vi "Pixelfly Example to Delete.vi"() -> ()   [LabVIEW 2016]
doc: "A short program to demonstrate the fundamentals of control and image acquision with the pco.camera series. The program records a sequence of images, with \"live\" updating, until the \"StopRecording\" button is pressed. Use ctrl-H for more help on the individual controls and indicators.\n\nCopyright 2004, 2010 The Cooke Corporation."
uses:
  pco.sdk/CameraAccess/CameraAccess.lvlib
  pco.sdk/ImageSensor/ImageSensor.lvlib
  pco.sdk/TimingControl/TimingControl.lvlib
  pco.recorder/Recorder.lvlib
  pco.sdk/RecordingControl/RecordingControl.lvlib
  pco.sdk/CameraDescription/CameraDescription.lvlib
panel:
  out "Recorded Images":u32=298
  in  "TriggerMode":u16(ring) items=["auto sequence"=0, "software trigger"=1, "external exposure start & software trigger"=2, "external exposure control"=3, "external synchronized"=4, "fast external exposure control"=5, "external CDS control"=6, "slow external exposure control"=7, "external synchronized HDSDI"=258]
  in  "Quit":bool
  out "Image":u16[][](graph)
  in  "Start Record":bool
  out "Recording On":bool
  in  "roiY1":u16=2048 min=2 max=2048 step=1
  in  "roiX1":u16=2048 min=2 max=2048 step=1
  in  "roiY0":u16=1 min=1 max=2047 step=1
  in  "roiX0":u16=1 min=1 max=2047 step=1
  out "Image Height":u16=2048
  out "Image Width":u16=2048
  in  "dwImgCount":u32=10 caption="Required Number of Images" max=5304
  in  "DelayTimeBase":u16(ring)=2 items=["nanoseconds", "microseconds", "milliseconds"]
  in  "ExposureTimeBase":u16(ring)=2 items=["nanoseconds", "microseconds", "milliseconds"]
  in  "Exposure":u32=100 min=1
  in  "Delay":u32
  in  "Rate":i32(ring) items=["Low", "High"]
  # "Camera Setup"
  # "Parameters for image readout"
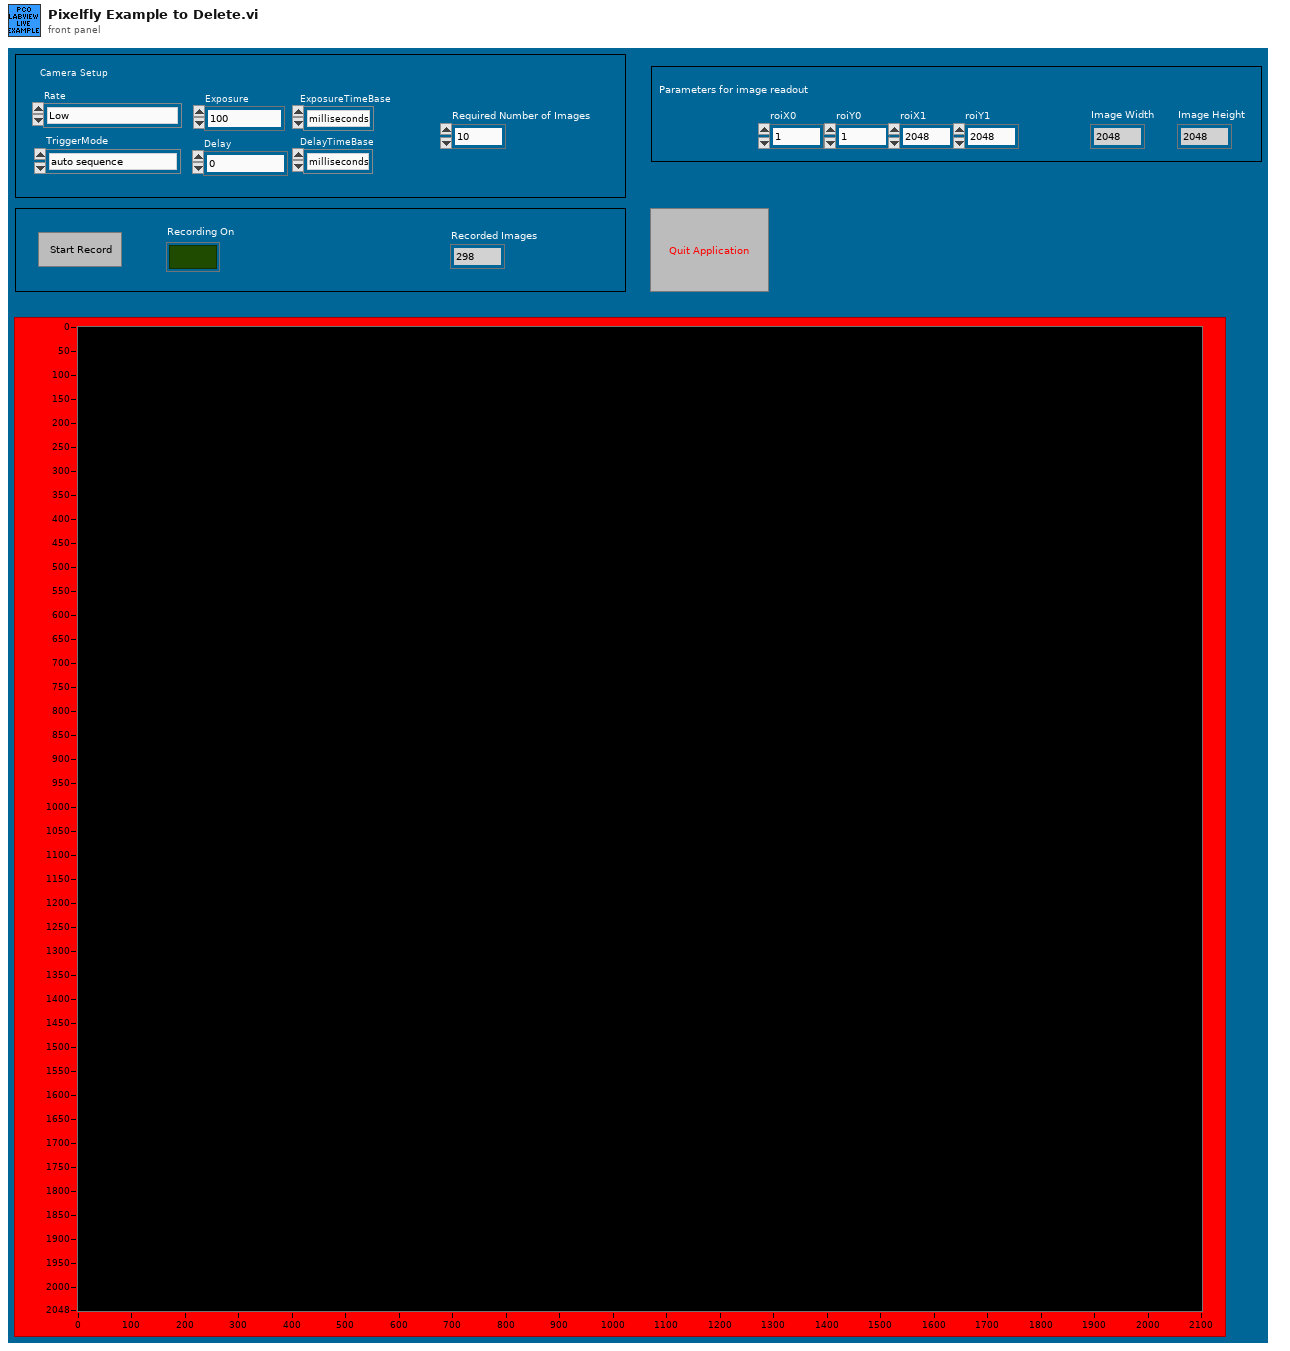
[diagram p1: front panel]
types:
  T1 = enum8{"Enabled", "Disabled", "Disabled and Grayed Out"}
  T2 = cluster{"wSensorTypeDESC":u16, "wSensorSubTypeDESC":u16, "wMaxHorzResStdDESC":u16, "wMaxVertResStdDESC":u16, "wMaxHorzResExtDESC":u16, "wMaxVertResExtDESC":u16, "wDynResDESC":u16, "wMaxBinHorzDESC":u16, "wBinHorzSteppingDESC":u16, "wMaxBinVertDESC":u16, "wBinVertSteppingDESC":u16, "wRoiHorStepsDESC":u16, "wRoiVertStepsDESC":u16, "wNumADCsDESC":u16, "wMinSizeHorzDESC":u16, "dwPixelRateDESC":u32[], "wConvFactDESC":u16[], "sCoolingSetpoints":i16[], "wSoftRoiHorStepsDESC":u16, "wSoftRoiVertStepsDESC":u16, "wIRDESC":u16, "wMinSizeVertDESC":u16, "dwMinDelayDESC":u32, "dwMaxDelayDESC":u32, "dwMinDelayStepDESC":u32, "dwMinExposureDESC":u32, "dwMaxExposureDESC":u32, "dwMinExposureStepDESC":u32, "dwMinDelayIRDESC":u32, "dwMaxDelayIRDESC":u32, "dwMinExposureIRDESC":u32, "dwMaxExposureIRDESC":u32, "wTimeTableDESC":u16, "wDoubleImageDESC":u16, "sMinCoolSetDESC":i16, "sMaxCoolSetDESC":i16, "sDefaultCoolSetDESC":i16, "wPowerDownModeDESC":u16, "wOffsetRegulationDESC":u16, "wColorPatternDESC":u16, "wPatternTypeDESC":u16, "wNumCoolingSetpoints":u16, "dwGeneralCapsDESC1":u32, "dwGeneralCapsDESC2":u32, "dwExtSyncFrequency":u32[], "dwGeneralCapsDESC3":u32, "dwGeneralCapsDESC4":u32}
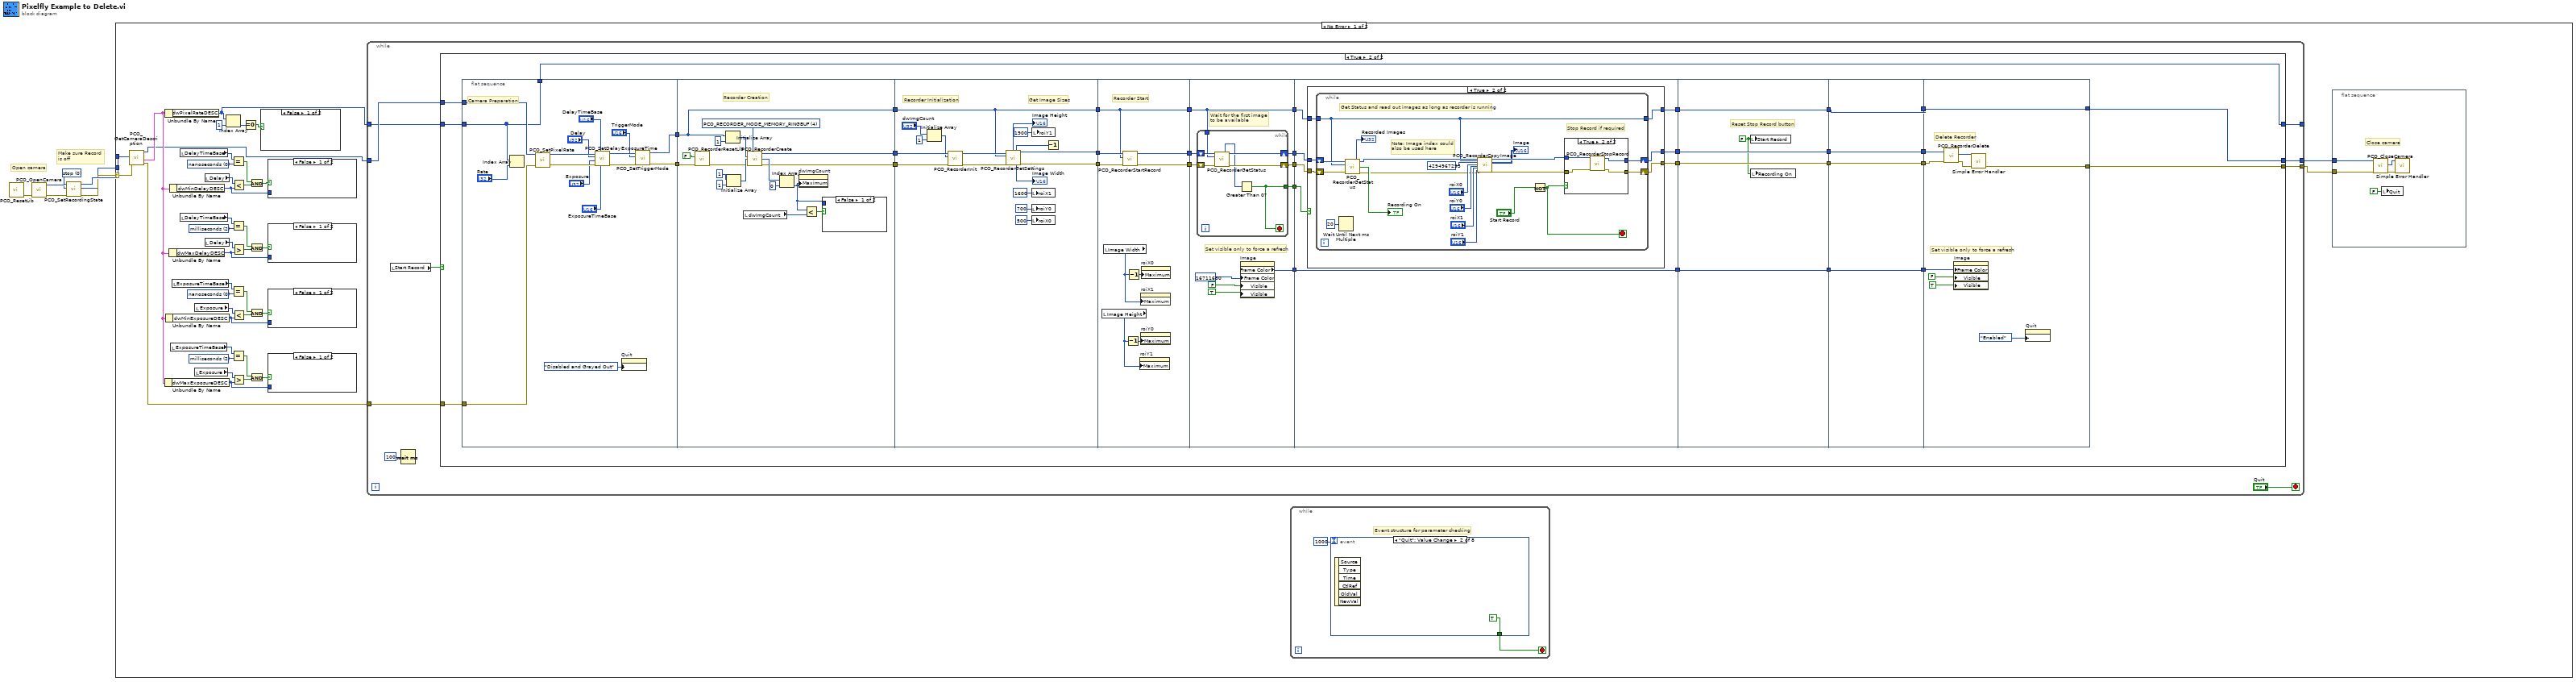
[diagram p0: block diagram]
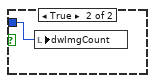
[diagram p3: hidden frame]
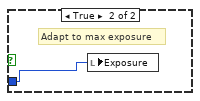
[diagram p6: hidden frame]
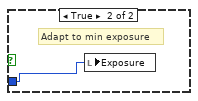
[diagram p7: hidden frame]
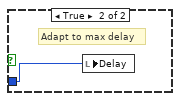
[diagram p8: hidden frame]
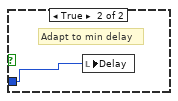
[diagram p9: hidden frame]
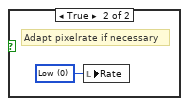
[diagram p10: hidden frame]
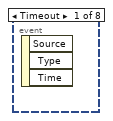
[diagram p11: hidden frame]
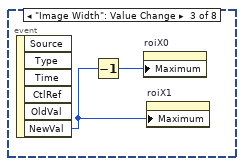
[diagram p12: hidden frame]
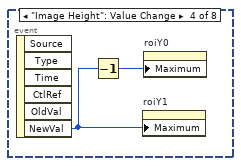
[diagram p13: hidden frame]
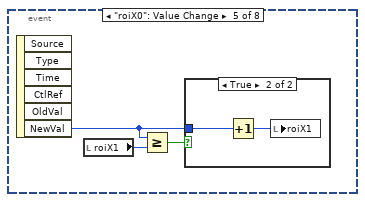
[diagram p14: hidden frame]
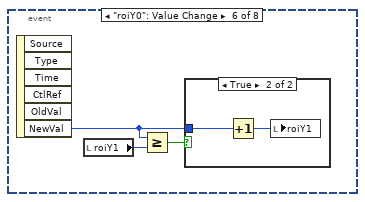
[diagram p16: hidden frame]
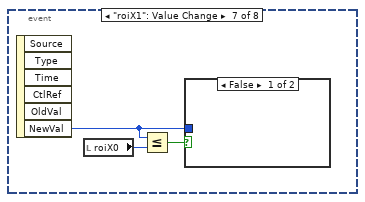
[diagram p18: hidden frame]
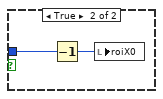
[diagram p19: hidden frame]
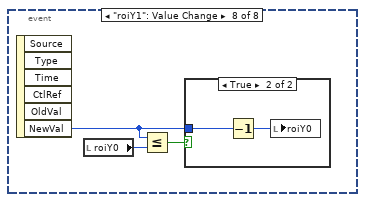
[diagram p20: hidden frame]
diagram:
  w4 = u16 0 items=["stop", "run"] ("wRecState")
  # "Make sure Record \nis off"
  # "Open camera"
  n1 = call "PCO_ResetLib.vi"() -> ("error out"=w7:errorcluster)  [unwired: 10 in, 1 out]
  n2 = call "PCO_OpenCamera.vi"("error in (no error)"=w7) -> ("error out"=w6:errorcluster, "ph out"=w5:u64)  [unwired: 8 in, 1 out]
  n3 = call "PCO_SetRecordingState.vi"("error in (no error)"=w6, "wRecState"=w4, "ph"=w5) -> ("error out"=w2:errorcluster, "ErrorMessage"=w1:i32, "ph out"=w3:u64)  [unwired: 6 in]
  n4 = case shown="No Error" w2 {
    selector: w2 -> [w14 w270]
    tunnel: w3 -> [w12 _]
    tunnel: w1 -> [_ w269]
    frame No Error {
      w35 = u16 2 items=["nanoseconds", "microseconds", "milliseconds"] ("DelayTimeBase")
      w44 = u16 0 items=["nanoseconds", "microseconds", "milliseconds"] ("DelayTimeBase")
      w28 = u16 2 items=["nanoseconds", "microseconds", "milliseconds"] ("DelayTimeBase")
      w19 = u16 0 items=["nanoseconds", "microseconds", "milliseconds"] ("DelayTimeBase")
      n5 = call "PCO_GetCameraDescription.vi"("error in (no error)"=w14, "ph"=w12) -> ("error out"=w13:errorcluster, "strDescription"=w46:T2, "ph out"=w11:u64)  [unwired: 6 in, 1 out]
      n6 = Unbundle By Name(w46) -> ("dwMaxExposureDESC"=w32:u32)
      n7 = Unbundle By Name(w46) -> ("dwPixelRateDESC"=w8:u32[])
      n8 = Unbundle By Name(w46) -> ("dwMinExposureDESC"=w39:u32)
      n9 = Unbundle By Name(w46) -> ("dwMaxDelayDESC"=w31:u32)
      n10 = Unbundle By Name(w46) -> ("dwMinDelayDESC"=w24:u32)
      n11 = local read "ExposureTimeBase"() -> (w36:u16)
      n12 = local read "ExposureTimeBase"() -> (w43:u16)
      n13 = local read "DelayTimeBase"() -> (w20:u16)
      n14 = local read "DelayTimeBase"() -> (w27:u16)
      n15 = local read "Exposure"() -> (w34:u32)
      n16 = local read "Exposure"() -> (w45:u32)
      n17 = local read "Delay"() -> (w18:u32)
      n18 = local read "Delay"() -> (w29:u32)
      n19 = Index Array(array=w8, index=1) -> (element=w16:u32)
      n20 = Equal?(x=w20, y=w19) -> (x = y?=w23:bool)
      n21 = Equal?(x=w27, y=w28) -> (x = y?=w25:bool)
      n22 = Equal?(x=w43, y=w44) -> (x = y?=w40:bool)
      n23 = Equal?(x=w36, y=w35) -> (x = y?=w38:bool)
      n24 = Less?(x=w18, y=w24) -> (x < y?=w22:bool)
      n25 = Greater?(x=w29, y=w31) -> (0:w26:bool)
      n26 = Less?(x=w45, y=w39) -> (x < y?=w41:bool)
      n27 = Greater?(x=w34, y=w32) -> (0:w37:bool)
      n28 = Equal To 0?(x=w16) -> (x = 0?=w17:bool)
      n29 = And(x=w23, y=w22) -> (x .and. y?=w21:bool)
      n30 = And(x=w25, y=w26) -> (x .and. y?=w30:bool)
      n31 = And(x=w40, y=w41) -> (x .and. y?=w42:bool)
      n32 = And(x=w38, y=w37) -> (x .and. y?=w33:bool)
      n33 = case shown="False" w17 {
        frame False {
        }
        frame True {
          w241 = 0 items=["Low", "High"] ("Rate")
          # "Adapt pixelrate if necessary"
          n34 = local write "Rate"(w241) -> ()
        }
      }
      n35 = case shown="False" w21 {
        tunnel: w24 -> [_ w240]
        frame False {
        }
        frame True {
          # "Adapt to min delay"
          n36 = local write "Delay"(w240) -> ()
        }
      }
      n37 = case shown="False" w30 {
        tunnel: w31 -> [_ w239]
        frame False {
        }
        frame True {
          # "Adapt to max delay"
          n38 = local write "Delay"(w239) -> ()
        }
      }
      n39 = case shown="False" w42 {
        tunnel: w39 -> [_ w238]
        frame False {
        }
        frame True {
          # "Adapt to min exposure"
          n40 = local write "Exposure"(w238) -> ()
        }
      }
      n41 = case shown="False" w33 {
        tunnel: w32 -> [_ w237]
        frame False {
        }
        frame True {
          # "Adapt to max exposure"
          n42 = local write "Exposure"(w237) -> ()
        }
      }
      n43 = while {
        tunnel: w13 -> [w60]
        tunnel: [w56] -> w9
        tunnel: w8 -> [w55]
        tunnel: [w54] -> _
        tunnel: w11 -> [w59]
        tunnel: [w58] -> w10
        stop <- "Quit" stop-if-true
        n44 = local read "Start Record"() -> (w57:bool)
        n45 = Wait (ms)(milliseconds to wait=u32 100) -> ()  [unwired: 1 out]
        n46 = case shown="True" w57 {
          tunnel: w60 -> [w63 w71]
          tunnel: w59 -> [w62 w70]
          tunnel: [w62 w69] -> w58
          tunnel: [w63 w66] -> w56
          tunnel: w55 -> [w61 w65]
          tunnel: [w61 w64] -> w54
          frame False {
          }
          frame True {
            n47 = flat-sequence {
              tunnel: [w103] -> w97
              tunnel: [w104] -> w96
              tunnel: w71 -> [w101]
              tunnel: w70 -> [w100]
              tunnel: w65 -> [w99]
              tunnel: [w99] -> w64
              tunnel: w97 -> [w129]
              tunnel: w96 -> [w117]
              tunnel: [w119] -> w95
              tunnel: [w118] -> w94
              tunnel: [w117] -> w93
              tunnel: w95 -> [w148]
              tunnel: w94 -> [w147]
              tunnel: [w138] -> w92
              tunnel: [w139] -> w91
              tunnel: w93 -> [w137]
              tunnel: [w137] -> w90
              tunnel: w92 -> [w157]
              tunnel: w91 -> [w156]
              tunnel: [w155] -> w89
              tunnel: [w154] -> w88
              tunnel: w90 -> [w153]
              tunnel: [w153] -> w87
              tunnel: w89 -> [w162]
              tunnel: [w160] -> w86
              tunnel: w88 -> [w163]
              tunnel: [w161] -> w85
              tunnel: w87 -> [w159]
              tunnel: [w159] -> w84
              tunnel: [w164] -> w83
              tunnel: [w158] -> w82
              tunnel: w86 -> [w182]
              tunnel: w85 -> [w180]
              tunnel: w84 -> [w181]
              tunnel: [w179] -> w81
              tunnel: [w178] -> w80
              tunnel: [w177] -> w79
              tunnel: w83 -> [w176]
              tunnel: [w176] -> w78
              tunnel: w82 -> [w175]
              tunnel: [w222] -> w77
              tunnel: w81 -> [w222]
              tunnel: [w221] -> w76
              tunnel: w80 -> [w221]
              tunnel: [w220] -> w75
              tunnel: w79 -> [w220]
              tunnel: w78 -> [w219]
              tunnel: [w219] -> w74
              tunnel: w77 -> [w224]
              tunnel: w76 -> [w223]
              tunnel: w75 -> [w225]
              tunnel: [w225] -> w73
              tunnel: [w226] -> w72
              tunnel: w74 -> [w226]
              tunnel: [w224] -> w68
              tunnel: [w223] -> w67
              tunnel: w73 -> [w231]
              tunnel: w72 -> [w232]
              tunnel: [w231] -> w69
              tunnel: w68 -> [w230]
              tunnel: w67 -> [w229]
              tunnel: [w228] -> w66
              frame #0 {
                # "Camera Preparation"
                n48 = Index Array(array=w99, index="Rate") -> ()  [unwired: 1 out]
                n49 = call "PCO_SetPixelRate.vi"("error in (no error)"=w101, "ph"=w100) -> ("error out"=w111:errorcluster, "ph out"=w112:u64)  [unwired: 7 in, 1 out]
                n50 = call "PCO_SetDelayExposureTime.vi"("wTimeBaseExposure"="ExposureTimeBase", "wTimeBaseDelay"="DelayTimeBase", "error in (no error)"=w111, "dwExposure"="Exposure", "dwDelay"="Delay", "ph"=w112) -> ("error out"=w105:errorcluster, "ph out"=w106:u64)  [unwired: 3 in, 1 out]
                n51 = property on="Quit" class="Bool (strict)"("DisabledEnum"=T1."Disabled and Grayed Out" ("Disabled")) -> ()  [unwired: 2 in, 2 out]
                n52 = call "PCO_SetTriggerMode.vi"("error in (no error)"=w105, "wTriggerMode"="TriggerMode", "ph"=w106) -> ("error out"=w103:errorcluster, "ph out"=w104:u64)  [unwired: 6 in, 1 out]
              }
              frame #1 {
                w126 = u32 4 items=["PCO_RECORDER_MODE_FILE"=1, "PCO_RECORDER_MODE_MEMORY_SEQUENCE"=2, "PCO_RECORDER_MODE_MEMORY_RINGBUF"=4, "PCO_RECORDER_MODE_MEMORY_FIFO"=8] ("dwRecMode")
                # "Recorder Creation"
                n53 = call "PCO_RecorderResetLib.vi"("error in (no error)"=w129, "bSilent"=FALSE) -> ("error out"=w120:errorcluster)  [unwired: 8 in, 1 out]
                n54 = Initialize Array(w117, 1 ("dimension size")) -> (w127:u64[])
                n55 = Initialize Array(u32 1 ("dimension size"), 1 ("dimension size")) -> (w123:u32[])
                n56 = local read "dwImgCount"() -> (w114:u32)
                n57 = call "PCO_RecorderCreate.vi"("dwRecMode"=w126, "phCamArr"=w127, "dwImgDistributionArr"=w123, "error in (no error)"=w120) -> ("phRec out"=w118:u64, "dwMaxImgCountArr"=w122:u32[], "error out"=w119:errorcluster)  [unwired: 8 in, 1 out]
                n58 = Index Array(array=w122, index=0) -> (element=w115:u32)
                n59 = property on="dwImgCount" class="DigNum (strict)"("Maximum"=w115) -> ()  [unwired: 2 in, 2 out]
                n60 = Less?(x=w115, y=w114) -> (x < y?=w116:bool)
                n61 = case shown="False" w116 {
                  tunnel: w115 -> [_ w131]
                  frame False {
                  }
                  frame True {
                    n62 = local write "dwImgCount"(w131) -> ()
                  }
                }
              }
              frame #2 {
                # "Get Image Sizes"
                # "Recorder Initialization"
                n63 = Initialize Array("dwImgCount", 1 ("dimension size")) -> (w144:u32[])
                n64 = call "PCO_RecorderInit.vi"("error in (no error)"=w148, "dwImgCountArr"=w144, "phRec"=w147) -> ("error out"=w143:errorcluster, "phRec out"=w142:u64)  [unwired: 6 in, 1 out]
                n65 = call "PCO_RecorderGetSettings.vi"("phRec"=w142, "phCam"=w137, "error in (no error)"=w143) -> ("wHeight"=→"Image Height":u16, "dwReqImgCount"=w134:u32, "phRec out"=w138:u64, "wWidth"=→"Image Width":u16, "error out"=w139:errorcluster)  [unwired: 4 in, 4 out]
                n66 = local write "roiX1"(u16 1600 ("roiX1")) -> ()
                n67 = local write "roiY0"(u16 700 ("roiY0")) -> ()
                n68 = local write "roiX0"(u16 500 ("roiY0")) -> ()
                n69 = local write "roiY1"(u16 1900 ("roiY1")) -> ()
                n70 = Decrement(x=w134) -> ()  [unwired: 1 out]
              }
              frame #3 {
                # "Recorder Start"
                n71 = local read "Image Height"() -> (w150:u16)
                n72 = local read "Image Width"() -> (w149:u16)
                n73 = call "PCO_RecorderStartRecord.vi"("error in (no error)"=w156, "phCam"=w153, "phRec"=w157) -> ("error out"=w155:errorcluster, "phRec out"=w154:u64)  [unwired: 6 in, 1 out]
                n74 = Decrement(x=w150) -> (x-1=w151:u16)
                n75 = Decrement(x=w149) -> (x-1=w152:u16)
                n76 = property on="roiY1" class="DigNum (strict)"("Maximum"=w150) -> ()  [unwired: 2 in, 2 out]
                n77 = property on="roiX1" class="DigNum (strict)"("Maximum"=w149) -> ()  [unwired: 2 in, 2 out]
                n78 = property on="roiY0" class="DigNum (strict)"("Maximum"=w151) -> ()  [unwired: 2 in, 2 out]
                n79 = property on="roiX0" class="DigNum (strict)"("Maximum"=w152) -> ()  [unwired: 2 in, 2 out]
              }
              frame #4 {
                # "Set visible only to force a refresh"
                # "Wait for the first image \nto be available"
                n80 = while {
                  shift-right: [w171] -> w160
                  shift-left: w162 -> [w172]
                  shift-right: [w173] -> w161
                  shift-left: w163 -> [w174]
                  tunnel: w159 -> [w169]
                  tunnel: [w168] -> w158
                  stop <- w168 stop-if-true
                  n81 = call "PCO_RecorderGetStatus.vi"("phRec"=w174, "phCam"=w169, "error in (no error)"=w172) -> ("dwProcImgCount"=w170:u32, "phRec out"=w173:u64, "error out"=w171:errorcluster)  [unwired: 2 in, 8 out]
                  n82 = Greater Than 0?(x=w170) -> (x > 0?=w168:bool)
                }
                n83 = property on="Image" class="IntGraph (strict)"("Frame Color"=u32 16711680, "Visible"=FALSE, "Visible"=TRUE) -> ("Frame Color"=w164:u32)  [unwired: 2 in, 2 out]
              }
              frame #5 {
                n84 = case shown="True" w175 {
                  tunnel: w182 -> [w183 w191]
                  tunnel: w181 -> [w185 w190]
                  tunnel: w180 -> [w184 w189]
                  tunnel: [w184 w188] -> w179
                  tunnel: [w183 w187] -> w178
                  tunnel: [w185 w186] -> w177
                  frame False {
                    # "Skip readout if nothing has been recorded"
                  }
                  frame True {
                    n85 = while {
                      tunnel: w190 -> [w197]
                      shift-right: [w198] -> w187
                      shift-left: w191 -> [w211]
                      shift-right: [w199] -> w188
                      shift-left: w189 -> [w202]
                      tunnel: [w197] -> w186
                      stop <- w193 stop-if-true
                      # "Note: Image index could \nalso be used here"
                      # "Stop Record if required"
                      # "Get Status and read out images as long as recorder is running"
                      n86 = Wait Until Next ms Multiple(millisecond multiple=u32 20) -> ()  [unwired: 1 out]
                      n87 = call "PCO_RecorderGetStatus.vi"("phRec"=w202, "phCam"=w197, "error in (no error)"=w211) -> ("dwProcImgCount"=→"Recorded Images":u32, "phRec out"=w209:u64, "bIsRunning"=→"Recording On":bool, "error out"=w203:errorcluster)  [unwired: 2 in, 7 out]
                      n88 = call "PCO_RecorderCopyImage.vi"("phRec"=w209, "phCam"=w197, "dwImgIdx"=u32 4294967295, "wRoiX0"="roiX0", "wRoiY0"="roiY0", "wRoiX1"="roiX1", "wRoiY1"="roiY1", "error in (no error)"=w203) -> ("phRec out"=w201:u64, "wImgBuf"=→"Image":u16[][], "error out"=w200:errorcluster)  [unwired: 13 in, 4 out]
                      n89 = Not(x="Start Record") -> (.not. x?=w193:bool)
                      n90 = case shown="True" w193 {
                        tunnel: w201 -> [w213 w217]
                        tunnel: w200 -> [w212 w216]
                        tunnel: [w213 w214] -> w199
                        tunnel: [w212 w215] -> w198
                        frame False {
                        }
                        frame True {
                          n91 = call "PCO_RecorderStopRecord.vi"("error in (no error)"=w216, "phRec"=w217) -> ("error out"=w215:errorcluster, "phRec out"=w214:u64)  [unwired: 7 in, 1 out]
                        }
                      }
                    }
                  }
                }
              }
              frame #6 {
                w218 = FALSE ("Stop Record")
                # "Reset Stop Record button"
                n92 = local write "Start Record"(w218) -> ()
                n93 = local write "Recording On"(w218) -> ()
              }
              frame #7 {
              }
              frame #8 {
                # "Set visible only to force a refresh"
                # "Delete Recorder"
                n94 = call "PCO_RecorderDelete.vi"("error in (no error)"=w229, "phRec"=w230) -> ("error out"=w235:errorcluster, "ErrorMessage"=w236:i32)  [unwired: 8 in]
                n95 = property on="Image" class="IntGraph (strict)"("Frame Color"=w232, "Visible"=FALSE, "Visible"=TRUE) -> ()  [unwired: 2 in, 2 out]
                n96 = call <vilib>:"Simple Error Handler.vi"("error code (no error:0)"=w236, "error in (no error)"=w235) -> ("error out"=w228:errorcluster)  [unwired: 3 in, 4 out]
                n97 = property on="Quit" class="Bool (strict)"("DisabledEnum"=T1."Enabled" ("Disabled")) -> ()  [unwired: 2 in, 2 out]
              }
            }
          }
        }
      }
      n98 = while {
        stop <- w242 stop-if-true
        # "Event structure for parameter checking"
        n99 = event shown="[1] \"Quit\": Value Change" {
          selector: _ -> [_ _ _ _ _ _ _ _]
          dyn-events: _ -> [_ _ _ _ _ _ _ _]
          timeout: 1000 -> [_ _ _ _ _ _ _ _]
          tunnel: [_ TRUE _ _ _ _ _ _] -> w242
          event Timeout {
            n100 = event-data() -> ()  [unwired: 1 in, 3 out]
          }
          event "Quit": Value Change {
            n101 = event-data() -> ()  [unwired: 1 in, 6 out]
          }
          event "Image Width": Value Change {
            n102 = event-data() -> ("NewVal"=w245:u16)  [unwired: 1 in, 5 out]
            n103 = Decrement(x=w245) -> (x-1=w246:u16)
            n104 = property on="roiX0" class="DigNum (strict)"("Maximum"=w246) -> ()  [unwired: 2 in, 2 out]
            n105 = property on="roiX1" class="DigNum (strict)"("Maximum"=w245) -> ()  [unwired: 2 in, 2 out]
          }
          event "Image Height": Value Change {
            n106 = event-data() -> ("NewVal"=w247:u16)  [unwired: 1 in, 5 out]
            n107 = Decrement(x=w247) -> (x-1=w248:u16)
            n108 = property on="roiY1" class="DigNum (strict)"("Maximum"=w247) -> ()  [unwired: 2 in, 2 out]
            n109 = property on="roiY0" class="DigNum (strict)"("Maximum"=w248) -> ()  [unwired: 2 in, 2 out]
          }
          event "roiX0": Value Change {
            n110 = event-data() -> ("NewVal"=w249:u16)  [unwired: 1 in, 5 out]
            n111 = local read "roiX1"() -> (w251:u16)
            n112 = Greater Or Equal?(x=w249, y=w251) -> (x >= y?=w250:bool)
            n113 = case shown="True" w250 {
              tunnel: w249 -> [_ w253]
              frame False {
              }
              frame True {
                n114 = Increment(x=w253) -> (x+1=w252:u16)
                n115 = local write "roiX1"(w252) -> ()
              }
            }
          }
          event "roiY0": Value Change {
            n116 = event-data() -> ("NewVal"=w254:u16)  [unwired: 1 in, 5 out]
            n117 = local read "roiY1"() -> (w256:u16)
            n118 = Greater Or Equal?(x=w254, y=w256) -> (x >= y?=w255:bool)
            n119 = case shown="True" w255 {
              tunnel: w254 -> [_ w258]
              frame False {
              }
              frame True {
                n120 = Increment(x=w258) -> (x+1=w257:u16)
                n121 = local write "roiY1"(w257) -> ()
              }
            }
          }
          event "roiX1": Value Change {
            n122 = event-data() -> ("NewVal"=w259:u16)  [unwired: 1 in, 5 out]
            n123 = local read "roiX0"() -> (w261:u16)
            n124 = Less Or Equal?(x=w259, y=w261) -> (x <= y?=w260:bool)
            n125 = case shown="False" w260 {
              tunnel: w259 -> [_ w263]
              frame False {
              }
              frame True {
                n126 = Decrement(x=w263) -> (x-1=w262:u16)
                n127 = local write "roiX0"(w262) -> ()
              }
            }
          }
          event "roiY1": Value Change {
            n128 = event-data() -> ("NewVal"=w264:u16)  [unwired: 1 in, 5 out]
            n129 = local read "roiY0"() -> (w266:u16)
            n130 = Less Or Equal?(x=w264, y=w266) -> (x <= y?=w265:bool)
            n131 = case shown="True" w265 {
              tunnel: w264 -> [_ w268]
              frame False {
              }
              frame True {
                n132 = Decrement(x=w268) -> (x-1=w267:u16)
                n133 = local write "roiY0"(w267) -> ()
              }
            }
          }
        }
      }
      n134 = flat-sequence {
        tunnel: w10 -> [w49]
        tunnel: w9 -> [w48]
        frame #0 {
          # "Close camera"
          n135 = call "PCO_CloseCamera.vi"("error in (no error)"=w48, "ph"=w49) -> ("error out"=w51:errorcluster, "ErrorMessage"=w50:i32)  [unwired: 8 in]
          n136 = local write "Quit"(FALSE ("Quit")) -> ()
          n137 = call <vilib>:"Simple Error Handler.vi"("error code (no error:0)"=w50, "error in (no error)"=w51) -> ()  [unwired: 3 in, 5 out]
        }
      }
    }
    frame Error {
      n138 = call <vilib>:"Simple Error Handler.vi"("error code (no error:0)"=w269, "error in (no error)"=w270) -> ()  [unwired: 3 in, 5 out]
    }
  }
